vi "RemoteVI Track Target.vi"(0 "state":T2, 5 "clients":T4(array[cluster]), 7 "context":T3) -> (4 "state out":T2, 6 "track":T1)   [LabVIEW 2020, in "RemoteVI.lvlib"]
doc: "One iteration of the server loop, first half: looks at the shared target. Loop Flags says what is due; Track Popups lists the LabVIEW popups (Win32 only) and Track Windows the application's other windows (leaving out the windows of other shares); a modal window or a disabled panel window counts as modal, modal or a popup as busy (no VI Server call then). Apply Splitter sets a bar a client dropped, Refresh Geometry refreshes the cached geometry, handle and origin when due, and after a refresh or a moved bar Read Panel Info reads the tip strips and splitter bars again. Returns the state with those updated and what it found (track) for Serve Clients Step."
uses:
  RemoteVI.lvlib
panel:
  in  "nothing tracked":T1
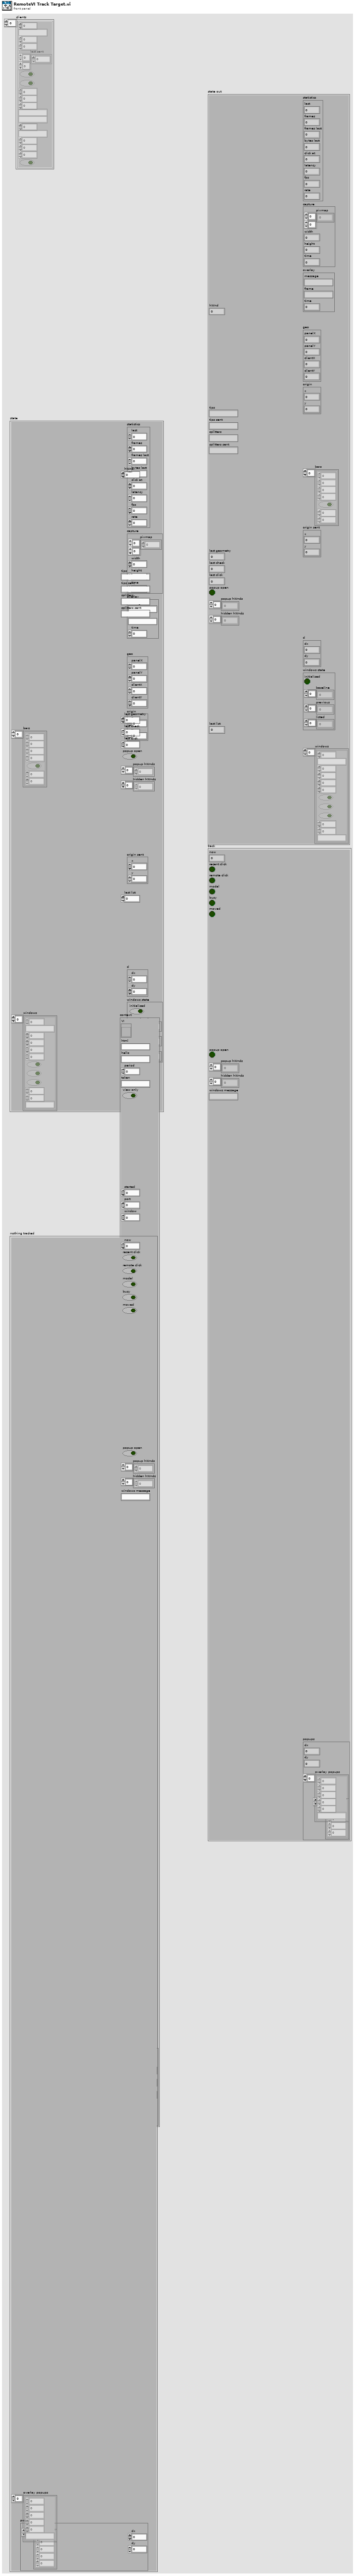
[diagram p1: front panel]
types:
  T1 = cluster{"now":u32, "recent click":bool, "remote click":bool, "modal":bool, "busy":bool, "moved":bool, "popups":cluster{"windows":cluster{"hwnd":u64, "x":i32, "y":i32, "w":i32, "h":i32}[], "dx":i32, "dy":i32}, "overlay popups":cluster{"hwnd":u64, "x":i32, "y":i32, "w":i32, "h":i32, "class":string}[], "popup open":bool, "popup hWnds":u64[], "hidden hWnds":u64[], "windows message":string}
  T2 = cluster{"statistics":cluster{"last":dbl, "frames":u32, "frames last":u32, "bytes last":dbl, "click at":dbl, "latency":dbl, "fps":dbl, "rate":dbl}, "capture":cluster{"pixmap":u32[][], "width":i32, "height":i32, "time":u32}, "overlay":cluster{"message":string, "frame":string, "time":u32}, "hWnd":u64, "geo":cluster{"panelX":i32, "panelY":i32, "clientX":i32, "clientY":i32}, "origin":cluster{"x":i32, "y":i32}, "tips":string, "tips sent":string, "splitters":string, "splitters sent":string, "bars":cluster{"x":i32, "y":i32, "w":i32, "h":i32, "vertical":bool, "min":i32, "max":i32}[], "origin sent":cluster{"x":i32, "y":i32}, "last geometry":u32, "last check":u32, "last click":u32, "popup open":bool, "popup hWnds":u64[], "hidden hWnds":u64[], "d":cluster{"dx":i32, "dy":i32}, "windows state":cluster{"initialised":bool, "baseline":u64[], "previous":u64[], "listed":u64[]}, "last list":u32, "windows":cluster{"id":u64, "title":string, "x":i32, "y":i32, "w":i32, "h":i32, "modal":bool, "active":bool, "closable":bool, "sx":i32, "sy":i32, "class":string}[]}
  T3 = cluster{"VI":refnum<vi>, "html":string, "hello":string, "period":dbl, "token":string, "view only":bool, "info":cluster{"port":u16, "url":string, "target":string, "kind":string, "whole network":bool, "view only":bool}, "started":dbl, "port":u16, "window":u64}
  T4 = cluster{"connection":u32, "rx buffer":string, "seq":u32, "acked":u32, "last sent":u32[][], "tracking":bool, "closed":bool, "mods":u8, "mods set":u8, "popup since":u32, "windows sent":string, "window frames":cluster{"id":u64, "pixels":u32[][]}[], "key window":u64, "address":string, "since":dbl, "last input":dbl, "bytes":dbl, "view only":bool}[]
  T5 = cluster{"panelX":i32, "panelY":i32, "clientX":i32, "clientY":i32}
  T6 = cluster{"x":i32, "y":i32, "w":i32, "h":i32, "vertical":bool, "min":i32, "max":i32}[]
  T7 = cluster{"initialised":bool, "baseline":u64[], "previous":u64[], "listed":u64[]}
  T8 = cluster{"id":u64, "title":string, "x":i32, "y":i32, "w":i32, "h":i32, "modal":bool, "active":bool, "closable":bool, "sx":i32, "sy":i32, "class":string}[]
  T9 = cluster{"windows":cluster{"hwnd":u64, "x":i32, "y":i32, "w":i32, "h":i32}[], "dx":i32, "dy":i32}
  T10 = cluster{"hwnd":u64, "x":i32, "y":i32, "w":i32, "h":i32, "class":string}[]
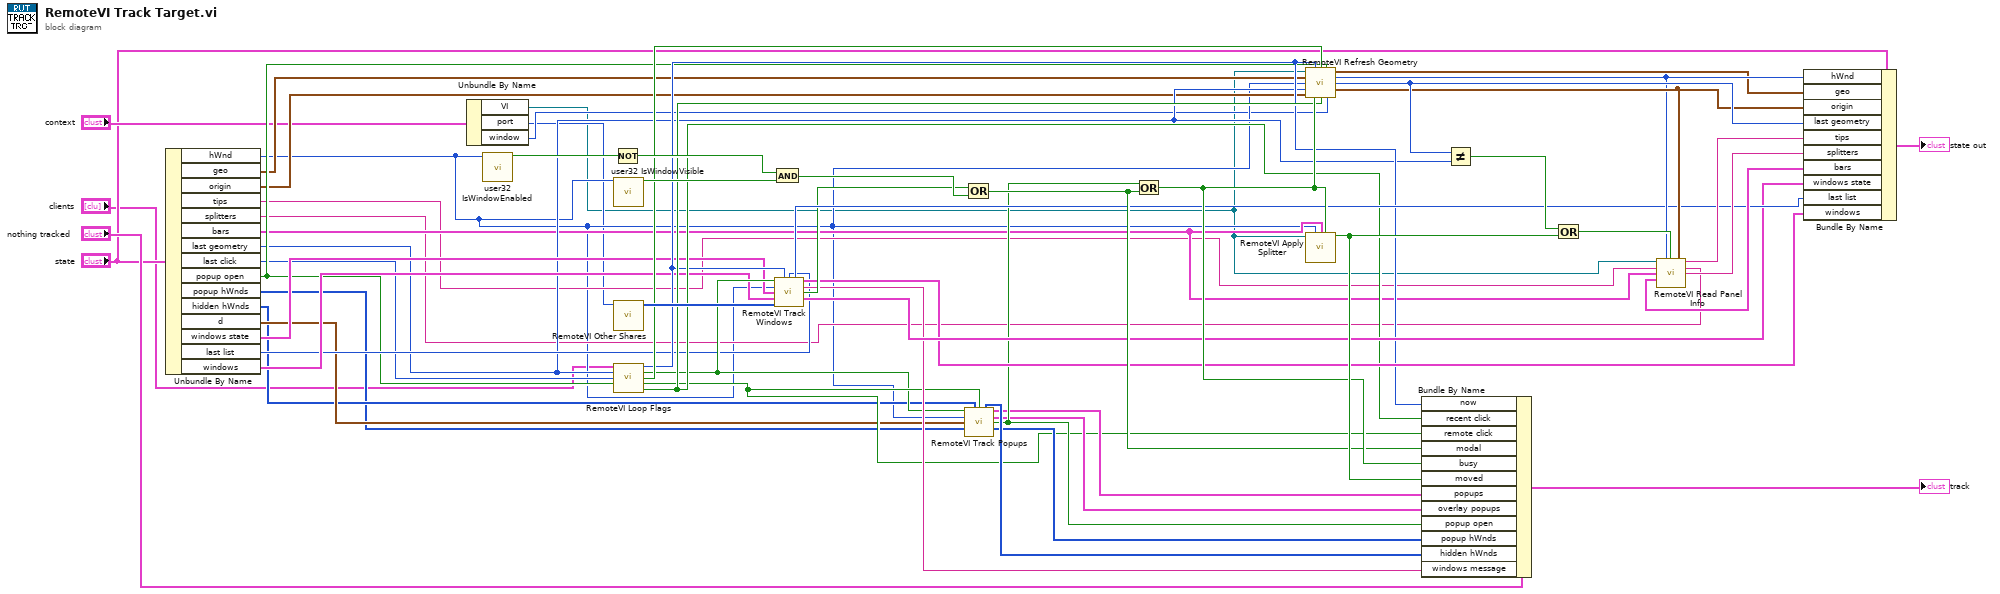
[diagram p0: block diagram]
diagram:
  n1 = Unbundle By Name("state") -> ("hWnd"=w7:u64, "geo"=w8:T5, "origin"=w9:cluster{"x":i32, "y":i32}, "tips"=w10:string, "splitters"=w11:string, "bars"=w12:T6, "last geometry"=w13:u32, "last click"=w14:u32, "popup open"=w15:bool, "popup hWnds"=w16:u64[], "hidden hWnds"=w17:u64[], "d"=w18:cluster{"dx":i32, "dy":i32}, "windows state"=w19:T7, "last list"=w20:u32, "windows"=w21:T8)
  n2 = Unbundle By Name("context") -> ("VI"=w4:refnum<vi>, "port"=w5:u16, "window"=w6:u64)
  n3 = call "user32 IsWindowEnabled.vi"("hWnd"=w7) -> ("enabled?"=w38:bool)  [unwired: 13 in, 1 out]
  n4 = Not(x=w38) -> (.not. x?=w40:bool)
  n5 = call "user32 IsWindowVisible.vi"("hWnd"=w7) -> ("visible?"=w39:bool)  [unwired: 13 in, 1 out]
  n6 = call "RemoteVI Other Shares.vi"("port"=w5) -> ("hWnds"=w32:u64[])  [unwired: 14 in]
  n7 = call "RemoteVI Loop Flags.vi"("clients"="clients", "last geometry"=w13, "last click"=w14, "popup was open?"=w15) -> ("now"=w22:u32, "look?"=w23:bool, "geometry due?"=w24:bool, "remote click?"=w25:bool, "recent click?"=w26:bool)  [unwired: 7 in]
  n8 = And(x=w40, y=w39) -> (x .and. y?=w41:bool)
  n9 = call "RemoteVI Track Windows.vi"("look?"=w23, "now"=w22, "last list"=w20, "panel hWnd"=w7, "state"=w19, "previous windows"=w21, "other shares"=w32) -> ("last list out"=w37:u32, "windows"=w33:T8, "message"=w34:string, "modal?"=w35:bool, "state out"=w36:T7)  [unwired: 4 in]
  n10 = Or(x=w35, y=w41) -> (x .or. y?=w42:bool)
  n11 = call "RemoteVI Track Popups.vi"("look?"=w23, "previously hidden"=w17, "remote click?"=w25, "panel hWnd"=w7, "d"=w18, "previous popup hWnds"=w16) -> ("hidden hWnds"=w31:u64[], "popups"=w27:T9, "overlay popups"=w28:T10, "popup open?"=w29:bool, "popup hWnds"=w30:u64[])  [unwired: 5 in]
  n12 = Or(x=w29, y=w42) -> (x .or. y?=w43:bool)
  n13 = call "RemoteVI Refresh Geometry.vi"("VI"=w4, "now"=w22, "geometry due?"=w24, "popup was open?"=w15, "geo"=w8, "hWnd"=w7, "last refresh"=w13, "origin"=w9, "popup open?"=w43, "recent click?"=w26, "window"=w6) -> ("geo out"=w45:T5, "hWnd out"=w46:u64, "last refresh out"=w48:u32, "origin out"=w47:cluster{"x":i32, "y":i32})  [unwired: 1 in]
  n14 = call "RemoteVI Apply Splitter.vi"("VI"=w4, "hWnd"=w7, "bars"=w12, "busy?"=w43) -> ("moved?"=w44:bool)  [unwired: 11 in]
  n15 = Bundle By Name(cluster="nothing tracked", "now"=w22, "recent click"=w26, "remote click"=w25, "modal"=w42, "busy"=w43, "moved"=w44, "popups"=w27, "overlay popups"=w28, "popup open"=w29, "popup hWnds"=w30, "hidden hWnds"=w31, "windows message"=w34) -> (→"track":T1)
  n16 = Not Equal?(x=w48, y=w13) -> (x != y?=w49:bool)
  n17 = Or(x=w49, y=w44) -> (x .or. y?=w50:bool)
  n18 = call "RemoteVI Read Panel Info.vi"("VI"=w4, "hWnd"=w46, "refresh?"=w50, "origin"=w47, "tips in"=w10, "splitters in"=w11, "bars in"=w12) -> ("tips out"=w51:string, "splitters out"=w52:string, "bars out"=w53:T6)  [unwired: 6 in]
  n19 = Bundle By Name(cluster="state", "hWnd"=w46, "geo"=w45, "origin"=w47, "last geometry"=w48, "tips"=w51, "splitters"=w52, "bars"=w53, "windows state"=w36, "last list"=w37, "windows"=w33) -> (→"state out":T2)
